vi "Page Explorer.vi"   [LabVIEW 2020]
types:
  T1 = enum32{"Invalid", "Standard", "Closed", "Hidden", "Minimized", "Maximized"}
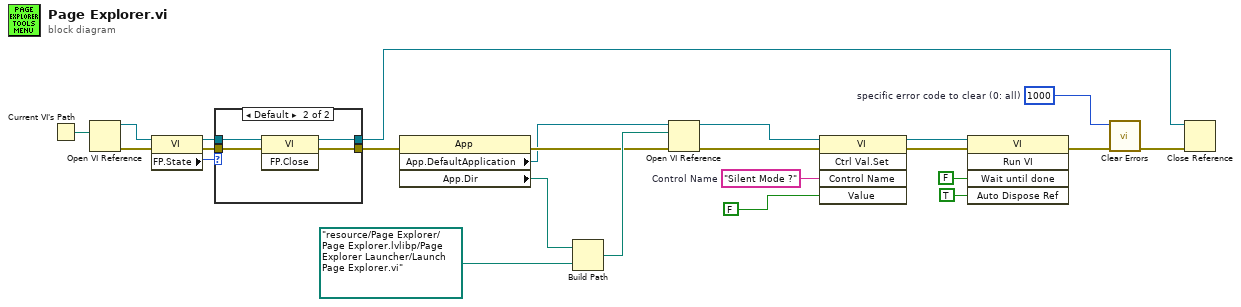
[diagram p0: block diagram]
diagram:
  w12 = 1000  # specific error code to clear (0: all)
  w16 = "Silent Mode ?"  # Control Name
  n1 = Current VI's Path() -> (path=w11:path)
  n2 = Open VI Reference(vi path=w11) -> (vi reference=w8:refnum<vi>, error out=w7:errorcluster)  [unwired: 5 in]
  n3 = property class="VI"(reference=w8, error in=w7) -> (reference out=w9:refnum<vi>, error out=w10:errorcluster, "FP.State"=w6:T1)
  n4 = case shown="Default" w6 {
    tunnel: [w26 w30] -> w5
    tunnel: w10 -> [w26 w29]
    tunnel: w9 -> [w25 w28]
    tunnel: [w25 w27] -> w4
    frame "Invalid", "Closed" {
    }
    frame Default {
      n5 = invoke class="VI" method="FP.Close"(reference=w28, error in=w29) -> (reference out=w27:refnum<vi>, error out=w30:errorcluster)  [unwired: 1 in, 1 out]
    }
  }
  n6 = property class="App"(error in=w5) -> (error out=w21:errorcluster, "App.DefaultApplication"=w3:refnum<vi>, "App.Dir"=w24:path)  [unwired: 1 in, 1 out]
  n7 = Build Path(base path=w24, name or relative path=path "resource/Page Explorer/Page Explorer.lvlibp/Page Explorer Launcher/Launch Page Explorer.vi" ("vi path")) -> (appended path=w22:path)
  n8 = Open VI Reference(application reference (local)=w3, vi path=w22, error in (no error)=w21) -> (vi reference=w14:refnum<vi>, error out=w13:errorcluster)  [unwired: 3 in]
  n9 = invoke class="VI" method="Ctrl Val.Set"(reference=w14, error in=w13, "Control Name"=w16, "Value"=FALSE ("Auto Dispose Reference")) -> (reference out=w17:refnum<vi>, error out=w18:errorcluster)  [unwired: 1 in, 3 out]
  n10 = invoke class="VI" method="Run VI"(reference=w17, error in=w18, "Wait until done"=FALSE ("Wait Until Done"), "Auto Dispose Ref"=TRUE ("Auto Dispose Reference")) -> (error out=w1:errorcluster)  [unwired: 1 in, 4 out]
  n11 = call <vilib>:"Clear Errors.vi"("error in (no error)"=w1, "specific error code to clear (0: all)"=w12) -> ("error out"=w2:errorcluster)  [unwired: 4 in, 1 out]
  n12 = Close Reference(reference=w4, error in (no error)=w2) -> ()  [unwired: 1 out]
